vi "CSE routine - build absolute path.vi"(4 "path in":path) -> (1 "path out":path)   [LabVIEW 2021]
doc: "::: CalcExpress Toolkit :::\nCopyright (c) 2000-2026 Konstantin Shifershteyn. All rights reserved."
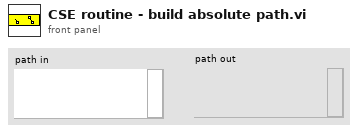
[diagram p1: front panel]
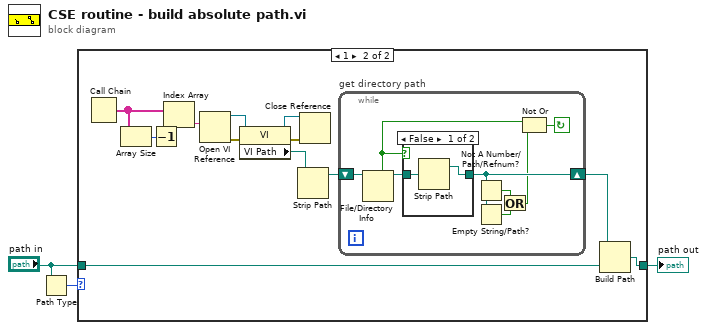
[diagram p0: block diagram]
diagram:
  n1 = Path Type(1:"path in") -> (0:w2:i16)
  n2 = case shown="1" w2 {
    tunnel: "path in" -> [w4 w9]
    tunnel: [w4 w7] -> w1
    frame 0, Default {
    }
    frame 1 {
      n3 = Call Chain() -> (call chain=w16:string[])
      n4 = Array Size(array=w16) -> (size(s)=w17:i32)
      n5 = Decrement(x=w17) -> (x-1=w15:i32)
      n6 = Index Array(array=w16, index=w15) -> (element=w14:string)
      n7 = Open VI Reference(vi path=w14) -> (vi reference=w13:refnum<vi>, error out=w12:errorcluster)  [unwired: 5 in]
      n8 = property on="Property Node" class="VI"(reference=w13, error in=w12) -> (reference out=w10:refnum<vi>, error out=w11:errorcluster, "VI Path"=w5:path)
      n9 = Strip Path(path=w5) -> (stripped path=w6:path)  [unwired: 1 out]
      n10 = Close Reference(reference=w10, error in (no error)=w11) -> ()  [unwired: 1 out]
      n11 = while "get directory path" {
        shift-left: w6 -> [w25]
        shift-right: [w23] -> w8
        stop <- w20 continue-if-true
        n12 = File/Directory Info(path=w25) -> (path out=w24:path, directory=w18:bool)  [unwired: 1 in, 5 out]
        n13 = case shown="False" w18 {
          tunnel: w24 -> [w27 w28]
          tunnel: [w26 w28] -> w23
          frame False {
            n14 = Strip Path(path=w27) -> (stripped path=w26:path)  [unwired: 1 out]
          }
          frame True {
          }
        }
        n15 = Not A Number/Path/Refnum?(number/path/refnum=w23) -> (NaN/Path/Refnum?=w21:bool)
        n16 = Empty String/Path?(string/path=w23) -> (empty?=w22:bool)
        n17 = Or(x=w21, y=w22) -> (x .or. y?=w19:bool)
        n18 = Not Or(1:w19, 2:w18) -> (0:w20:bool)
      }
      n19 = Build Path(base path=w8, name or relative path=w9) -> (appended path=w7:path)
    }
  }
  "path out" <- w1
